vi "CSM - Status Change Event.vi"(6 "Auto Register? (T)":bool=TRUE, 8 "Error In":errorcluster caption="error in (no error)", 9 "Wait (5000ms)":i32=5000, 11 "CSM Module":string) -> (0 "error out":errorcluster, 1 "Waited (ms)":u32, 3 "Status Change Event":refnum<user-event>)   [LabVIEW 2017, in "Communicable State Machine.lvlib"]
doc: "Obtains the CSM status change event refnum.\n\n-- <b>Controls</b> --\n- <b>CSM Module</b>: CSM module name.\n- <b>Wait (5000 ms)</b>: Timeout duration for waiting. The default is 5000 ms.\n\n-- <b>Indicators</b> --\n- <b>Status Change Event</b>: CSM status change event refnum.\n- <b>Waited (ms)</b>: Time elapsed while waiting."
uses:
  Communicable State Machine.lvlib
  _Support/Typedef/_CSM Status Change Event Data.ctl
  _Support/CSMQ/_CSMOFGVOPER.ctl
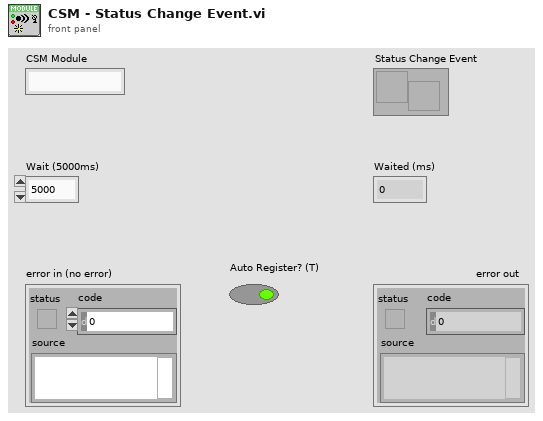
[diagram p1: front panel]
types:
  T1 = typedef "Communicable State Machine.lvlib/_CSMOFGVOPER.ctl" = enum16{"Create If not Exist", "Get By Name", "List", "Check If Name Exists", "Release", "Module Status", "Create Status Event Handler", "Destroy Status Event Handler", "Clear Invalid Objs"}
  T2 = typedef "Communicable State Machine.lvlib/_CSMObj.ctl" = cluster{"info":T3, "Refs":T5}
  T3 = typedef "Communicable State Machine.lvlib/_CSMObj-Info.ctl" = cluster{"Module Name":string, "Requested Name":string, "Group Name":string, "Mode":T4, "Allowed Messages":string[]}
  T4 = typedef "Communicable State Machine.lvlib/_CSM_MODE.ctl" = enum16{"Not Exist", "Stand Alone", "CSM", "Worker", "Worker Agent", "Chain Node", "Chain"}
  T5 = typedef "Communicable State Machine.lvlib/_CSMObj-Refs.ctl" = cluster{"WatchDogQ":refnum<queue>, "CSMDataDVR":refnum<data-value>, "Queue":T6, "GroupDataDVR":refnum<data-value>, "TagMap":refnum<data-value>, "ExitEvent":refnum<user-event>, "NewStateEvent":refnum<user-event>, "StatusEvent":refnum<user-event>, "InterruptEvent":refnum<user-event>}
  T6 = typedef "Communicable State Machine.lvlib/Priority Queue.ctl" = cluster{"HPriorityQ":refnum<queue>, "LowPriorityQ":refnum<queue>}
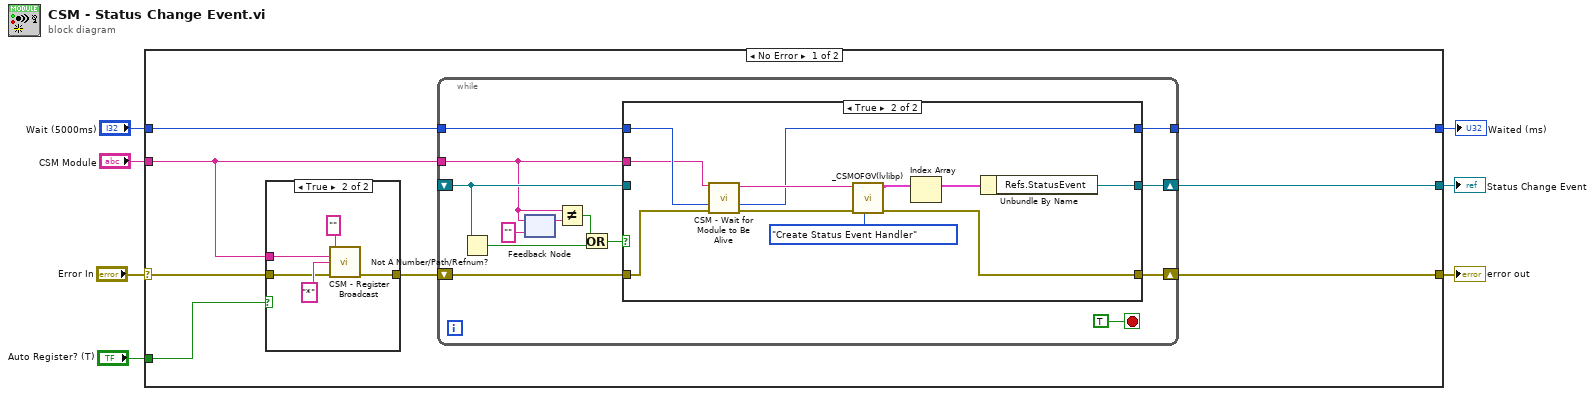
[diagram p0: block diagram]
diagram:
  n1 = case shown="No Error" "Error In" {
    selector: "Error In" -> [w11 w48]
    tunnel: [w15 _] -> w5
    tunnel: [w12 w48] -> w6
    tunnel: "CSM Module" -> [w9 _]
    tunnel: "Wait (5000ms)" -> [w14 _]
    tunnel: [w13 _] -> w2
    tunnel: "Auto Register? (T)" -> [w8 _]
    frame No Error {
      n2 = case shown="True" w8 {
        tunnel: w11 -> [w16 w19]
        tunnel: [w16 w18] -> w10
        tunnel: w9 -> [_ w17]
        frame False {
        }
        frame True {
          n3 = call "CSM - Register Broadcast.vi"("CSM Name(Empty for Broadcast Event)"="" ("CSM Name"), "Source CSM Name (* as Default)"=w17, "Trigger"="*" ("CSM Name"), "Error In"=w19) -> ("error out"=w18:errorcluster)  [unwired: 10 in, 1 out]
        }
      }
      n4 = while {
        shift-right: [w32] -> w12
        shift-left: w10 -> [w33]
        shift-right: [w34] -> w15
        shift-left: _ -> [w30]
        tunnel: w9 -> [w28]
        tunnel: w14 -> [w23]
        tunnel: [w22] -> w13
        stop <- TRUE stop-if-true
        n5 = Not A Number/Path/Refnum?(number/path/refnum=w30) -> (NaN/Path/Refnum?=w26:bool)
        n6 = feedback-in #1(w28) -> ()
        n7 = feedback #1("" ("CSM Module")) -> (w27:string)
        n8 = Not Equal?(x=w28, y=w27) -> (x != y?=w25:bool)
        n9 = Or(x=w25, y=w26) -> (x .or. y?=w29:bool)
        n10 = case shown="True" w29 {
          tunnel: [w36 w43] -> w34
          tunnel: w33 -> [w35 w42]
          tunnel: [w35 w46] -> w32
          tunnel: w30 -> [w36 _]
          tunnel: w28 -> [_ w38]
          tunnel: w23 -> [_ w39]
          tunnel: [_ w37] -> w22
          frame False {
          }
          frame True {
            n11 = call "CSM - Wait for Module to Be Alive.vi"("CSM Name"=w38, "Wait (5000 ms)"=w39, "error in (no error)"=w42) -> ("CSM Name (Dup)"=w40:string, "Waited (ms)"=w37:u32, "error out"=w41:errorcluster)  [unwired: 10 in]
            n12 = call "_CSMOFGV(lvlibp).vi"("Operation"=_CSMOFGVOPER."Create Status Event Handler", "Error In"=w41, "Name (\"\" to Use UUID) In"=w40) -> ("error out"=w46:errorcluster, "Array"=w45:T2[])  [unwired: 6 in, 1 out]
            n13 = Index Array(array=w45) -> (element=w44:T2)  [unwired: 1 in]
            n14 = Unbundle By Name(w44) -> ("Refs.StatusEvent"=w43:refnum<user-event>)
          }
        }
      }
    }
    frame Error {
    }
  }
  "error out" <- w6
  "Status Change Event" <- w5
  "Waited (ms)" <- w2
